vi "Conpane Caller.vi"() -> (0 "Result":dbl)   [LabVIEW 2026]
doc: "Round-13 end-to-end proof: a static Call to Conpane Probe B.vi, whose terminals exist ONLY because its AIXML carries conIdx. 3 * 5 must come back 15. If the connector pane were decoration, this would fail to link."
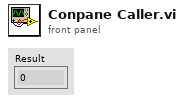
[diagram p1: front panel]
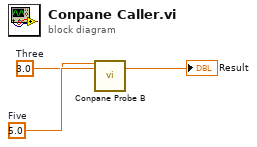
[diagram p0: block diagram]
diagram:
  w2 = 5.0  # Five
  w1 = 3.0  # Three
  n1 = call "Conpane Probe B.vi"("x"=w1, "factor"=w2) -> ("y"=→"Result":dbl)  [unwired: 13 in]
